vi "Generate Menu File.vi"(6 "Include Ancestor Palette ?":bool, 7 "Overwrite Always":bool, 8 "error in (no error)":errorcluster, 10 "Palette Fiole List":T7, 11 "Library as Project item":refnum<vi>) -> (0 "error out":errorcluster, 2 "palette data":T1={"display name"="", "view format"=0, "palette width"=4, "items"=[], "256 color icon"=bytes[0], "B&W color icon"=bytes[0], "help information"={"help tag"="", "help file path "=path ""}, "palette description"="", "synchronize information"={"synchronize with directory"=FALSE, "synchronize directory path"=path ""}} {"view format" items=["Icons", "Text", "Icons and Text"]}, 3 "Palette file path":path)   [LabVIEW 2012, in "Palette Generation.lvlib"]
doc: "This VI does most of the hard work, creating a palette file type def structure based on a list of project items that should belong in a virtual folder."
uses:
  Palette Generation.lvlib
  TypeDefs/Palette Fiole List.ctl
  <vilib>/Palette API/Palette Menu/Public Type Define/Palette Data.ctl
  <vilib>/Palette API/Palette Menu/Public Type Define/View Format.ctl
  <vilib>/Palette API/Palette Menu/Public Type Define/Items.ctl
  <vilib>/Palette API/Palette Menu/Public Type Define/Item.ctl
  <vilib>/Palette API/Palette Menu/Public Type Define/Help Info.ctl
  <vilib>/Palette API/Palette Menu/Public Type Define/Synchronize Info.ctl
  <vilib>/Palette API/Palette Menu/Public Type Define/Palette type.ctl
  <userlib>/_OpenG.lib/file/file.llb/File Exists - Scalar__ogtk.vi
  <userlib>/_OpenG.lib/file/file.llb/Strip Path Extension - String__ogtk.vi
  <userlib>/_OpenG.lib/file/file.llb/Convert File Extension (String)__ogtk.vi
  <userlib>/_OpenG.lib/file/file.llb/Strip Path Extension - Path__ogtk.vi
  <vilib>/regexp/Match Regular Expression.xnode
  <vilib>/Palette API/Palette Menu/Palette Menu.lvlib
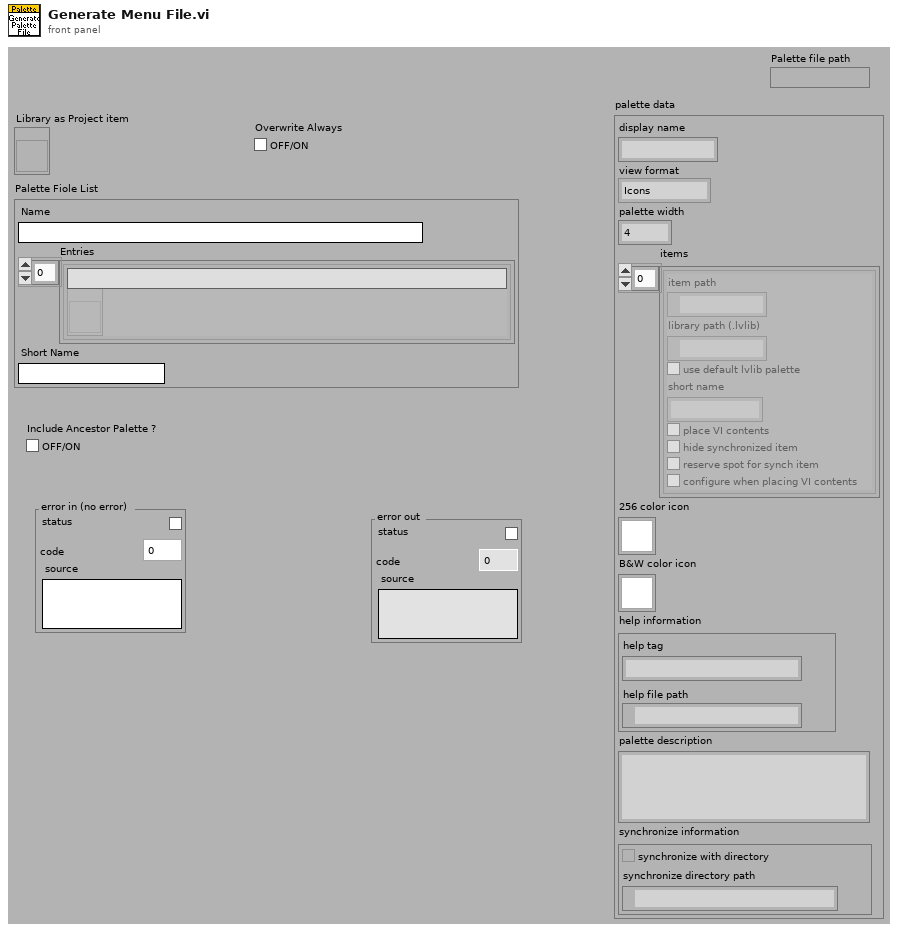
[diagram p1: front panel]
types:
  T1 = typedef "Palette Menu.lvlib/Palette Data.ctl" = cluster{"display name":string, "view format":T2, "palette width":i16, "items":T3, "256 color icon":picture, "B&W color icon":picture, "help information":T5, "palette description":string, "synchronize information":T6}
  T2 = typedef "Palette Menu.lvlib/View Format.ctl" = u16
  T3 = typedef "Palette Menu.lvlib/Items.ctl" = T4[]
  T4 = typedef "Palette Menu.lvlib/Item.ctl" = cluster{"item path":path, "library path (.lvlib)":path, "use default lvlib palette":bool, "short name":string, "place VI contents":bool, "hide synchronized item":bool, "reserve spot for synch item":bool, "configure when placing VI contents":bool}
  T5 = typedef "Palette Menu.lvlib/Help Info.ctl" = cluster{"help tag":string, "help file path ":path}
  T6 = typedef "Palette Menu.lvlib/Synchronize Info.ctl" = cluster{"synchronize with directory":bool, "synchronize directory path":path}
  T7 = typedef "Palette Generation.lvlib/Palette Fiole List.ctl" = cluster{"Name":string, "Entries":cluster{string, refnum<vi>}[], "Short Name":string}
  T8 = typedef "Palette Menu.lvlib/Palette type.ctl" = i32
  T9 = typedef "imagedata.ctl" = cluster{"image type":i32, "image depth":i32, "image":u8[], "mask":u8[], "colors":u32[], "Rectangle":cluster{"left":i16, "top":i16, "right":i16, "bottom":i16}}
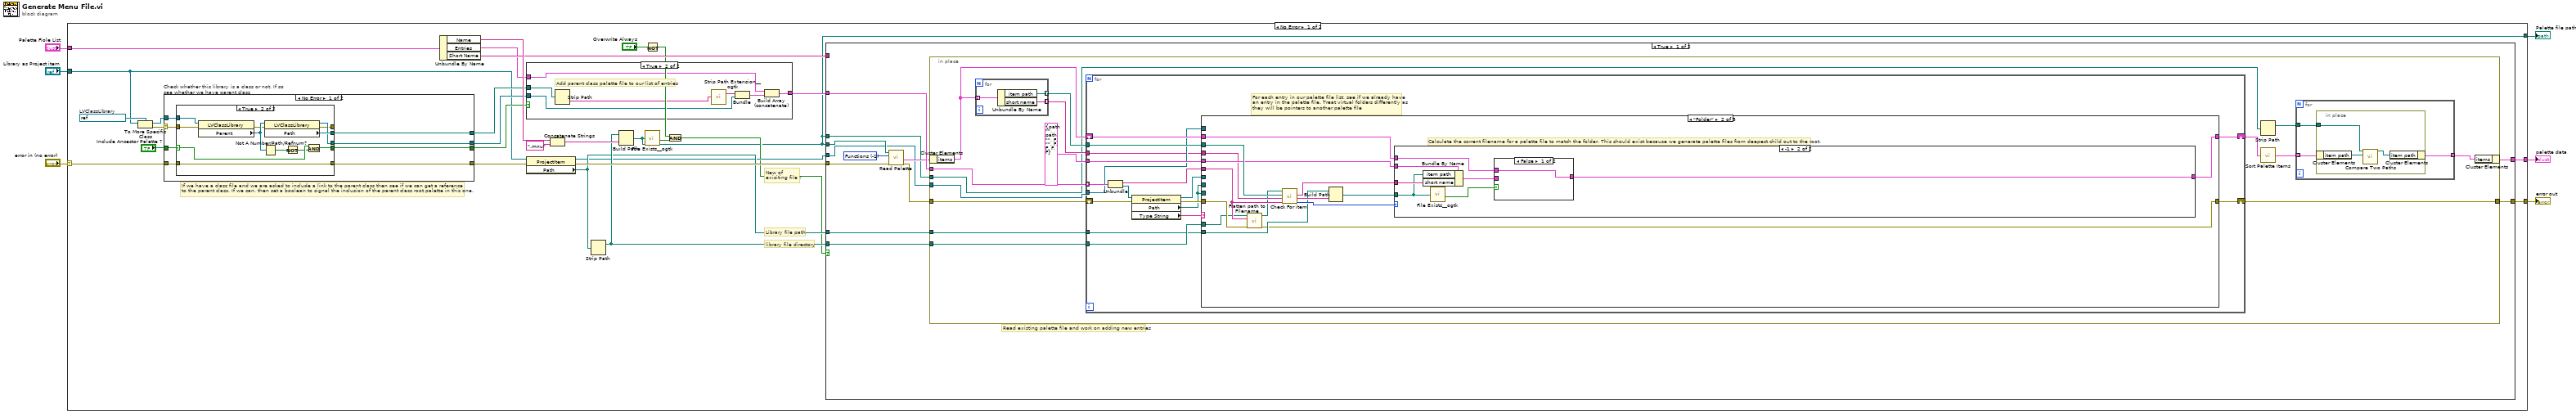
[diagram p0: block diagram]
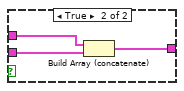
[diagram p7: hidden frame]
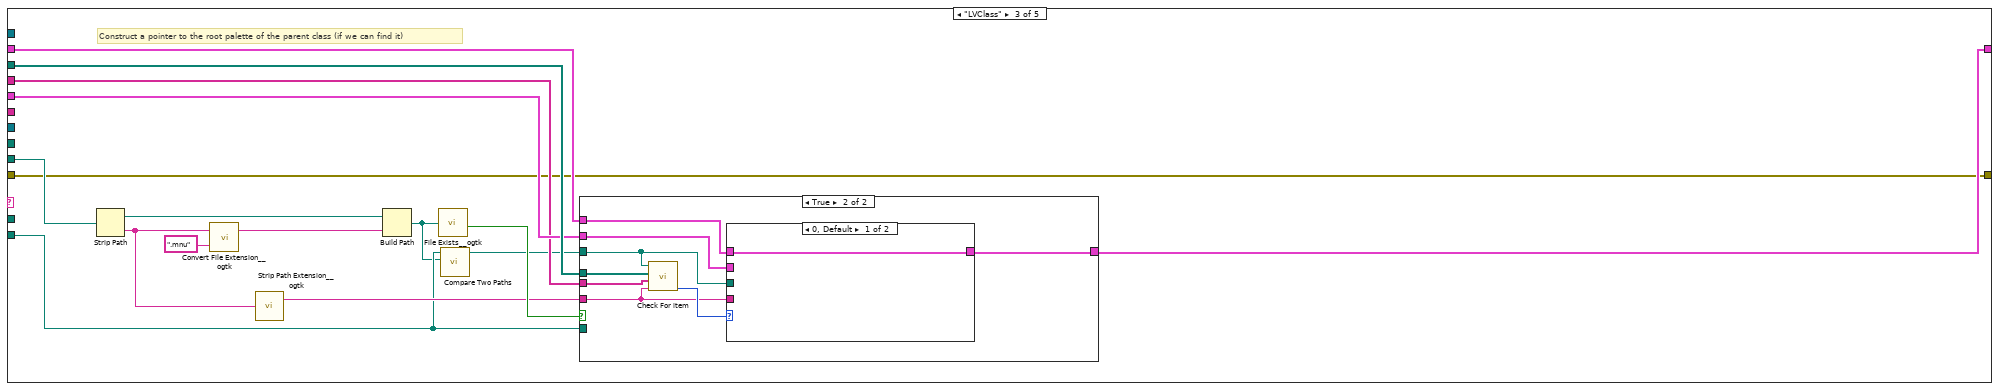
[diagram p8: hidden frame]
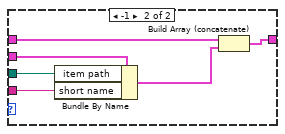
[diagram p10: hidden frame]
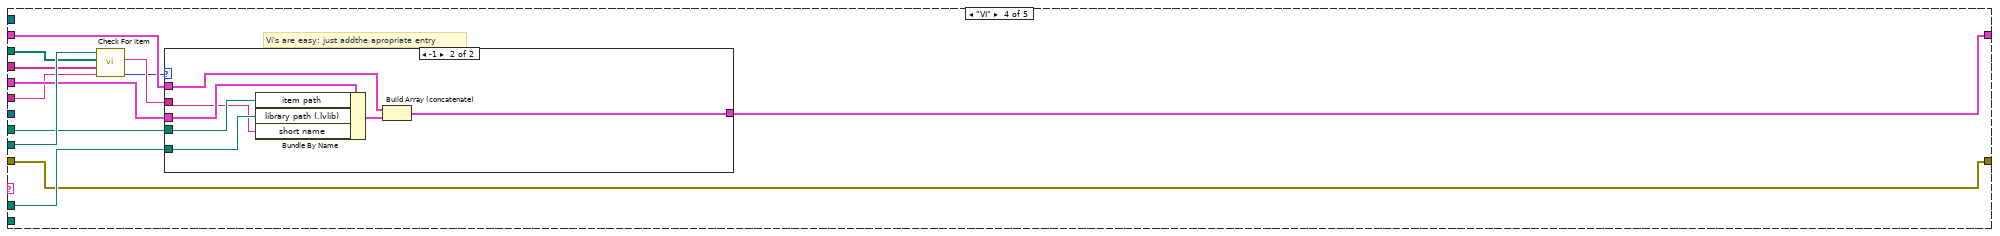
[diagram p11: hidden frame]
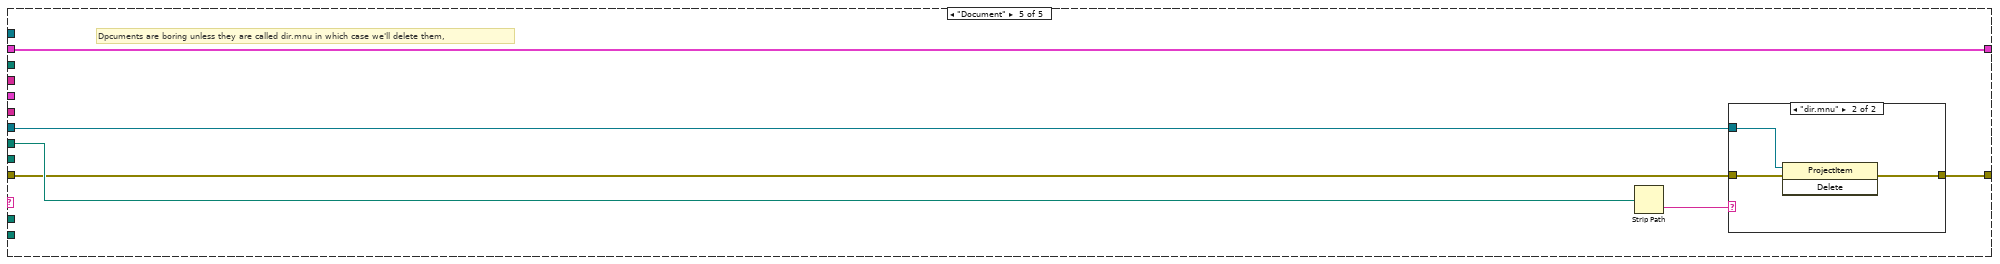
[diagram p13: hidden frame]
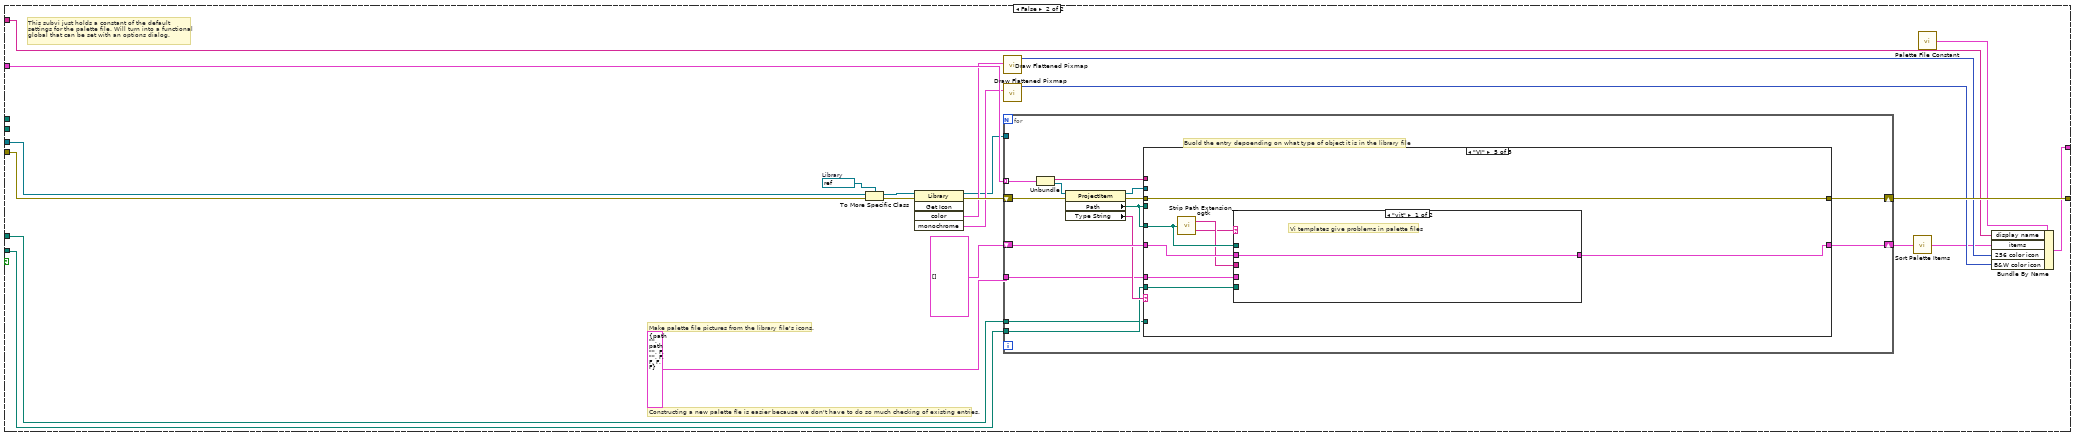
[diagram p15: hidden frame]
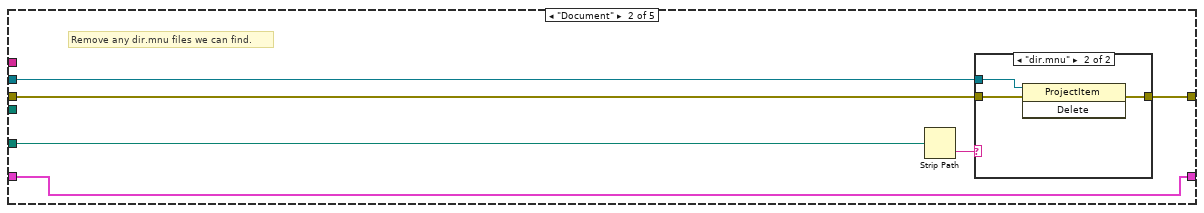
[diagram p17: hidden frame]
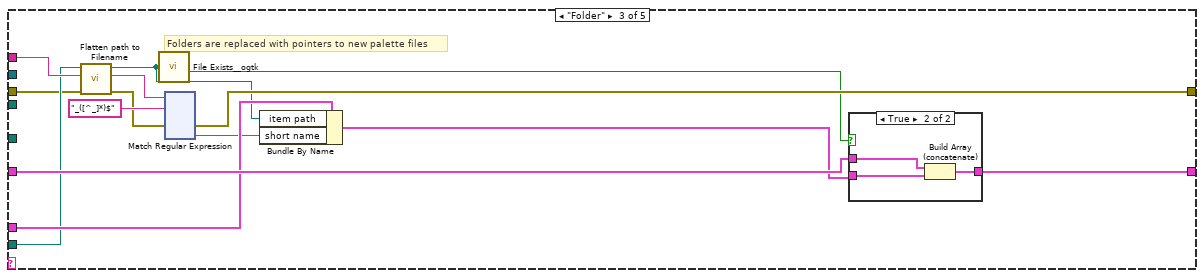
[diagram p19: hidden frame]
diagram:
  n1 = case shown="No Error" "error in (no error)" {
    selector: "error in (no error)" -> [w18 w425]
    tunnel: [w27 w425] -> w6
    tunnel: "Palette Fiole List" -> [w34 _]
    tunnel: "Library as Project item" -> [w9 _]
    tunnel: [w24 _] -> w2
    tunnel: [w7 _] -> w1
    frame No Error {
      w19 = refnum<vi> refnum  # LVClassLibrary
      # "New of\nexisiting file ?"
      # "library file directory"
      # "Library file path"
      # "If we have a class file and we are asked to include a link to the parent class then see if we can get a reference\nto the parent class. If we can, then set a boolean to signal the inclusion of the parent class root palette in this one."
      n2 = To More Specific Class(target class=w19, reference=w9) -> (specific class reference=w16:refnum<vi>, error out=w17:errorcluster)  [unwired: 1 in]
      n3 = case "Check whether this library is a class or not. If so see whether we have parent class" shown="No Error" w17 {
        selector: w17 -> [w49 _]
        tunnel: w18 -> [w43 w65]
        tunnel: w16 -> [w50 _]
        tunnel: [w47 _] -> w10
        tunnel: [w48 _] -> w11
        tunnel: [w46 w65] -> w15
        tunnel: [w44 _] -> w14
        tunnel: "Include Ancestor Palette ?" -> [w45 _]
        frame No Error {
          n4 = case shown="True" w45 {
            selector: w45 -> [w51 w60]
            tunnel: w50 -> [_ w64]
            tunnel: w49 -> [w52 w63]
            tunnel: [_ w62] -> w48
            tunnel: [_ w61] -> w47
            tunnel: [w52 w54] -> w46
            tunnel: [w51 w59] -> w44
            tunnel: w43 -> [_ w54]
            tunnel: [_ w53] -> _
            frame False {
            }
            frame True {
              n5 = property class="LVClassLibrary"(reference=w64, error in=w63) -> (error out=w55:errorcluster, "Parent"=w58:refnum<vi>)  [unwired: 1 out]
              n6 = Not A Number/Path/Refnum?(number/path/refnum=w58) -> (NaN/Path/Refnum?=w57:bool)
              n7 = property class="LVClassLibrary"(reference=w58, error in=w55) -> (reference out=w61:refnum<vi>, error out=w53:errorcluster, "Path"=w62:path)
              n8 = Not(x=w57) -> (.not. x?=w56:bool)
              n9 = And(x=w60, y=w56) -> (x .and. y?=w59:bool)
            }
          }
        }
        frame Error {
        }
      }
      n10 = Unbundle By Name(w34) -> ("Name"=w25:string, "Entries"=w12:cluster{string, refnum<vi>}[], "Short Name"=w23:string)
      n11 = case shown="True" w14 {
        tunnel: [w35 w41] -> w13
        tunnel: w12 -> [w35 w42]
        tunnel: w11 -> [_ w39]
        tunnel: w10 -> [_ w36]
        frame False {
        }
        frame True {
          # "Add parent class palette file to our list of entries"
          n12 = Strip Path(path=w39) -> (name=w40:string)  [unwired: 1 out]
          n13 = call-poly <userlib>:"Strip Path Extension__ogtk.vi"("path"=w40) -> ("root"=w37:string)  [unwired: 1 out]
          n14 = Bundle("root"=w37, "Parent"=w36) -> (w38:cluster{"root":string, "Parent":refnum<vi>})  [unwired: 1 out]
          n15 = Build Array (concatenate)(w42, w38) -> (w41:cluster{"root":string, "Parent":refnum<vi>}[])
        }
      }
      n16 = property class="ProjectItem"(reference=w9, error in=w15) -> (reference out=w26:refnum<vi>, error out=w30:errorcluster, "Path"=w28:path)
      n17 = Concatenate Strings(w25, ".mnu" ("string")) -> (w32:string)
      n18 = Strip Path(path=w28) -> (stripped path=w29:path)  [unwired: 1 out]
      n19 = Build Path(base path=w29, name or relative path=w32) -> (appended path=w7:path)
      n20 = call-poly <userlib>:"File Exists__ogtk.vi"("file path"=w7) -> ("exists"=w31:bool)  [unwired: 6 in, 1 out]
      n21 = Not(x="Overwrite Always") -> (.not. x?=w20:bool)
      n22 = And(x=w20, y=w31) -> (x .and. y?=w22:bool)
      n23 = case shown="True" w22 {
        tunnel: w7 -> [w77 _]
        tunnel: w30 -> [w75 w224]
        tunnel: w13 -> [w74 w233]
        tunnel: w29 -> [w72 w231]
        tunnel: w28 -> [w71 w230]
        tunnel: [w70 w229] -> w27
        tunnel: [w68 w226] -> w24
        tunnel: w26 -> [w67 w223]
        tunnel: w23 -> [_ w217]
        tunnel: w7 -> [w66 _]
        frame True {
          w76 = T8 -1 items=["Functions"=-1, "Controls"=-2] ("palette type")
          # "Read existing palette file and work on adding new entries"
          n24 = call <vilib>:"Read Palette.vi"("error in (no error)"=w75, "palette type"=w76, "palette path"=w77) -> ("error out"=w73:errorcluster, "palette data"=w69:T1)  [unwired: 1 in, 6 out]
          n25 = in-place {
            in-place-border: w74 -> [w92]
            in-place-border: w73 -> [w91]
            in-place-border: w72 -> [w89]
            in-place-border: w71 -> [w88]
            in-place-border: [w87] -> w70
            in-place-border: w67 -> [w86]
            in-place-border: w66 -> [w81]
            n26 = in-place-cluster #1(w69) -> ("items"=w85:T3)
            n27 = for {
              tunnel: w85 -> [w101] mode=indexing
              tunnel: [w100] -> w84 mode=indexing
              tunnel: [w99] -> w83 mode=indexing
              n28 = Unbundle By Name(w101) -> ("item path"=w100:path, "short name"=w99:string)
            }
            n29 = for {
              tunnel: w92 -> [w118] mode=indexing
              shift-right: [w107] -> w87
              shift-left: w91 -> [w116]
              tunnel: w84 -> [w115]
              shift-right: [w113] -> w82
              shift-left: w85 -> [w114]
              tunnel: T4 {"item path"=path "", "library path (.lvlib)"=path "", "use default lvlib palette"=FALSE, "short name"="", "place VI contents"=FALSE, "hide synchronized item"=FALSE, "reserve spot for synch item"=FALSE, "configure when placing VI contents"=FALSE} ("Items") -> [w110]
              tunnel: w89 -> [w109]
              tunnel: w88 -> [w108]
              tunnel: w86 -> [w104]
              tunnel: w83 -> [w102]
              # "For each entry in our palette file list, see if we already have\nan entry in the palette file. Treat virtual folders differently as\nthey will be pointers to another palette file"
              n30 = Unbundle(w118) -> ("root"=w111:string, "Parent"=w117:refnum<vi>)
              n31 = property class="ProjectItem"(reference=w117, error in=w116) -> (reference out=w103:refnum<vi>, error out=w106:errorcluster, "Path"=w105:path, "Type String"=w112:string)
              n32 = case shown="\"Folder\"" w112 {
                selector: w112 -> [w120 _ _ _ _]
                tunnel: w105 -> [w119 _ w160 w193 _]
                tunnel: w115 -> [_ w137 w165 w192 _]
                tunnel: w114 -> [w122 w134 w163 w191 w204]
                tunnel: [w122 w135 w164 w190 w204] -> w113
                tunnel: w111 -> [_ w127 _ w186 _]
                tunnel: w110 -> [_ w133 w162 w189 _]
                tunnel: w109 -> [_ w123 _ w187 _]
                tunnel: w108 -> [_ w128 w152 _ _]
                tunnel: [w121 w125 w154 w185 w203] -> w107
                tunnel: w106 -> [w121 w126 w154 w185 w205]
                tunnel: w105 -> [_ _ _ w188 w206]
                tunnel: w104 -> [_ _ _ _ _]
                tunnel: w103 -> [_ _ _ _ w202]
                tunnel: w102 -> [_ w131 w161 w184 _]
                frame "False", Default {
                  # "Ignore anything we don't recognise"
                  n33 = stacked-sequence {
                    tunnel: w120 -> [_]
                    tunnel: w119 -> [_]
                    frame #0 {
                    }
                  }
                }
                frame "Folder" {
                  # "Calculate the corrent filename for a palette file to match the folder. This should exist because we generate palette files from deepest child out to the root."
                  n34 = call "Flatten path to Filename.vi"("error in (no error)"=w126, "Virtual Folder's Virtual Path"=w127, "Library Base Path"=w123) -> ("error out"=w125:errorcluster, "Palette Path"=w124:path)  [unwired: 6 out]
                  n35 = call "Check For item.vi"("This Name"=w127, "short names"=w131, "item paths"=w137, "This Path"=w124) -> ("index of element"=w136:i32, "Flattened Name"=w129:string, "Short Name"=w132:string)  [unwired: 5 out]
                  n36 = Build Path(base path=w128, name or relative path=w129) -> (appended path=w130:path)
                  n37 = case shown="-1" w136 {
                    tunnel: [w138 w144] -> w135
                    tunnel: w134 -> [w138 w145]
                    tunnel: w133 -> [_ w143]
                    tunnel: w130 -> [_ w140]
                    tunnel: w132 -> [_ w142]
                    frame 0, Default {
                    }
                    frame -1 {
                      n38 = Bundle By Name(cluster=w143, "item path"=w140, "short name"=w142) -> (w141:T4)
                      n39 = call-poly <userlib>:"File Exists__ogtk.vi"("file path"=w140) -> ("exists"=w139:bool)  [unwired: 6 in, 1 out]
                      n40 = case shown="False" w139 {
                        tunnel: w145 -> [w146 w149]
                        tunnel: [w146 w148] -> w144
                        tunnel: w141 -> [_ w147]
                        frame False {
                        }
                        frame True {
                          n41 = Build Array (concatenate)(w149, w147) -> (w148:T3)
                        }
                      }
                    }
                  }
                }
                frame "LVClass" {
                  # "Construct a pointer to the root palette of the parent class (if we can find it)"
                  n42 = Strip Path(path=w160) -> (stripped path=w157:path, name=w156:string)
                  n43 = call-poly <userlib>:"Convert File Extension__ogtk.vi"("new ending (none)"=".mnu", "file name"=w156) -> ("new filename"=w158:string)  [unwired: 1 out]
                  n44 = call-poly <userlib>:"Strip Path Extension__ogtk.vi"("path"=w156) -> ("root"=w153:string)  [unwired: 1 out]
                  n45 = Build Path(base path=w157, name or relative path=w158) -> (appended path=w151:path)
                  n46 = call-poly <userlib>:"File Exists__ogtk.vi"("file path"=w151) -> ("exists"=w155:bool)  [unwired: 6 in, 1 out]
                  n47 = call <vilib>:"Compare Two Paths.vi"("Path 2"=w151, "Path 1"=w152) -> ("Relative Path from 1 to 2"=w150:path)  [unwired: 1 in, 8 out]
                  n48 = case shown="True" w155 {
                    tunnel: w165 -> [_ w174]
                    tunnel: [w166 w172] -> w164
                    tunnel: w163 -> [w166 w171]
                    tunnel: w162 -> [_ w170]
                    tunnel: w161 -> [_ w169]
                    tunnel: w152 -> [_ _]
                    tunnel: w153 -> [_ w167]
                    tunnel: w150 -> [_ w168]
                    frame False {
                    }
                    frame True {
                      n49 = call "Check For item.vi"("This Name"=w167, "short names"=w169, "item paths"=w174, "This Path"=w168) -> ("index of element"=w173:i32)  [unwired: 7 out]
                      n50 = case shown="0, Default" w173 {
                        tunnel: [w175 w180] -> w172
                        tunnel: w171 -> [w175 w181]
                        tunnel: w170 -> [_ w179]
                        tunnel: w168 -> [_ w178]
                        tunnel: w167 -> [_ w177]
                        frame 0, Default {
                        }
                        frame -1 {
                          n51 = Bundle By Name(cluster=w179, "item path"=w178, "short name"=w177) -> (w176:T4)
                          n52 = Build Array (concatenate)(w181, w176) -> (w180:T3)
                        }
                      }
                    }
                  }
                }
                frame "VI" {
                  # "Vi's are easy: just addthe apropriate entry"
                  n53 = call "Check For item.vi"("This Name"=w186, "short names"=w184, "item paths"=w192, "This Path"=w193) -> ("index of element"=w182:i32, "Short Name"=w183:string)  [unwired: 6 out]
                  n54 = case shown="-1" w182 {
                    tunnel: w191 -> [w194 w201]
                    tunnel: [w194 w200] -> w190
                    tunnel: w189 -> [_ w199]
                    tunnel: w188 -> [_ w197]
                    tunnel: w187 -> [_ w196]
                    tunnel: w183 -> [_ w195]
                    frame 0, Default {
                    }
                    frame -1 {
                      n55 = Bundle By Name(cluster=w199, "item path"=w197, "library path (.lvlib)"=w196, "short name"=w195) -> (w198:T4)
                      n56 = Build Array (concatenate)(w201, w198) -> (w200:T3)
                    }
                  }
                }
                frame "Document" {
                  # "Dpcuments are boring unless they are called dir.mnu in which case we'll delete them,"
                  n57 = Strip Path(path=w206) -> (name=w207:string)  [unwired: 1 out]
                  n58 = case shown="\"dir.mnu\"" w207 {
                    tunnel: w205 -> [w208 w211]
                    tunnel: w202 -> [_ w210]
                    tunnel: [w208 w209] -> w203
                    frame "False", Default {
                    }
                    frame "dir.mnu" {
                      n59 = invoke class="ProjectItem" method="Delete"(reference=w210, error in=w211) -> (error out=w209:errorcluster)  [unwired: 1 in, 2 out]
                    }
                  }
                }
              }
            }
            n60 = Strip Path(path=w81) -> (stripped path=w80:path)  [unwired: 1 out]
            n61 = call "Sort Palette Items.vi"("Array 2"=w82) -> ("Array"=w79:T4[])
            n62 = for {
              tunnel: w79 -> [w95] mode=indexing
              tunnel: w80 -> [w94]
              tunnel: [w93] -> w78 mode=indexing
              n63 = in-place {
                in-place-border: w94 -> [w97]
                n64 = in-place-cluster #2(w95) -> ("item path"=w98:path)
                n65 = call <vilib>:"Compare Two Paths.vi"("Path 2"=w98, "Path 1"=w97) -> ("Relative Path from 1 to 2"=w96:path)  [unwired: 1 in, 8 out]
                n66 = in-place-cluster #2("item path"=w96) -> (w93:T4)
              }
            }
            n67 = in-place-cluster #1("items"=w78) -> (w68:T1)
          }
        }
        frame False {
          w222 = refnum<vi> refnum  # Library
          # "This subvi just holds a constant of the default\nsettings for the palette file. Will turn into a functional\nglobal that can be set with an options dialog."
          # "Make palette file pictures from the library file's icons."
          # "Constructing a new palette fle is easier because we don't have to do so much checking of existing entries."
          n68 = To More Specific Class(target class=w222, reference=w223, error in=w224) -> (specific class reference=w221:refnum<vi>, error out=w220:errorcluster)
          n69 = invoke class="Library" method="Get Icon"(reference=w221, error in=w220) -> (reference out=w214:refnum<vi>, error out=w225:errorcluster, "color"=w219:T9, "monochrome"=w216:T9)  [unwired: 3 in, 1 out]
          n70 = call <vilib>:"Draw Flattened Pixmap.vi"("image data"=w219) -> ("new picture"=w218:picture)  [unwired: 1 in, 7 out]
          n71 = call <vilib>:"Draw Flattened Pixmap.vi"("image data"=w216) -> ("new picture"=w215:picture)  [unwired: 1 in, 7 out]
          n72 = for {
            tunnel: w233 -> [w247] mode=indexing
            shift-right: [w238] -> w229
            shift-left: w225 -> [w245]
            shift-right: [w243] -> w213
            shift-left: T4[] [] -> [w244]
            tunnel: T4 {"item path"=path "", "library path (.lvlib)"=path "", "use default lvlib palette"=FALSE, "short name"="", "place VI contents"=FALSE, "hide synchronized item"=FALSE, "reserve spot for synch item"=FALSE, "configure when placing VI contents"=FALSE} ("Items") -> [w241]
            tunnel: w231 -> [w240]
            tunnel: w230 -> [w239]
            tunnel: w214 -> [_]
            # "Buold the entry depoending on what type of object it is in the library file"
            n73 = Unbundle(w247) -> ("root"=w235:string, "Parent"=w246:refnum<vi>)
            n74 = property class="ProjectItem"(reference=w246, error in=w245) -> (reference out=w234:refnum<vi>, error out=w237:errorcluster, "Path"=w236:path, "Type String"=w242:string)
            n75 = case shown="\"VI\"" w242 {
              selector: w242 -> [w249 _ _ _ _]
              tunnel: w236 -> [_ _ _ w396 _]
              tunnel: w244 -> [w251 w253 w274 w405 w414]
              tunnel: [w251 w253 w275 w406 w413] -> w243
              tunnel: w241 -> [_ _ w273 w404 w412]
              tunnel: w240 -> [_ _ w266 _ w411]
              tunnel: w239 -> [_ _ _ w395 _]
              tunnel: [w250 w254 w270 w402 w408] -> w238
              tunnel: w237 -> [w250 w255 w265 w402 w408]
              tunnel: w236 -> [w248 w257 _ _ w410]
              tunnel: w235 -> [_ _ w268 _ _]
              tunnel: w234 -> [_ w252 _ _ _]
              frame "False", Default {
                # "An unknown type"
                n76 = stacked-sequence {
                  tunnel: w249 -> [_]
                  tunnel: w248 -> [_]
                  frame #0 {
                  }
                }
              }
              frame "Document" {
                # "Remove any dir.mnu files we can find."
                n77 = Strip Path(path=w257) -> (name=w256:string)  [unwired: 1 out]
                n78 = case shown="\"dir.mnu\"" w256 {
                  tunnel: w255 -> [w258 w261]
                  tunnel: w252 -> [_ w260]
                  tunnel: [w258 w259] -> w254
                  frame "False", Default {
                  }
                  frame "dir.mnu" {
                    n79 = invoke class="ProjectItem" method="Delete"(reference=w260, error in=w261) -> (error out=w259:errorcluster)  [unwired: 1 in, 2 out]
                  }
                }
              }
              frame "Folder" {
                # "Folders are replaced with pointers to new palette files"
                n80 = call "Flatten path to Filename.vi"("error in (no error)"=w265, "Virtual Folder's Virtual Path"=w268, "Library Base Path"=w266) -> ("error out"=w264:errorcluster, "result string"=w267:string, "Palette Path"=w263:path)  [unwired: 5 out]
                n81 = call-poly <userlib>:"File Exists__ogtk.vi"("file path"=w263) -> ("exists"=w262:bool)  [unwired: 6 in, 1 out]
                n82 = xnode "Match Regular Expression"("input string"=w267, "regular expression"="_([^_]*)$", "error in"=w264) -> ("error out"=w270:errorcluster, "submatch 1"=w269:string)  [unwired: 1 in, 6 out]
                n83 = Bundle By Name(cluster=w273, "item path"=w263, "short name"=w269) -> (w272:T4)
                n84 = case shown="True" w262 {
                  tunnel: [w276 w279] -> w275
                  tunnel: w274 -> [w276 w278]
                  tunnel: w272 -> [_ w277]
                  frame False {
                  }
                  frame True {
                    n85 = Build Array (concatenate)(w278, w277) -> (w279:T4[])
                  }
                }
              }
              frame "LVClass" {
                # "Classes are replaced with pointers to the root palette file if it exists. This is called when the parent class link is required."
                n86 = Strip Path(path=w396) -> (stripped path=w399:path, name=w400:string)
                n87 = call-poly <userlib>:"Strip Path Extension__ogtk.vi"("path"=w400) -> ("root"=w393:string)  [unwired: 1 out]
                n88 = call-poly <userlib>:"Convert File Extension__ogtk.vi"("new ending (none)"=".mnu", "file name"=w400) -> ("new filename"=w398:string)  [unwired: 1 out]
                n89 = Build Path(base path=w399, name or relative path=w398) -> (appended path=w401:path)
                n90 = call-poly <userlib>:"File Exists__ogtk.vi"("file path"=w401) -> ()  [unwired: 6 in, 2 out]
                n91 = call <vilib>:"Compare Two Paths.vi"("Path 2"=w401, "Path 1"=w395) -> ("Relative Path from 1 to 2"=w394:path)  [unwired: 1 in, 8 out]
                n92 = Bundle By Name(cluster=w404, "item path"=w394, "short name"=w393) -> (w403:T4)
                n93 = Build Array (concatenate)(w405, w403) -> (w406:T4[])
              }
              frame "VI" {
                n94 = call-poly <userlib>:"Strip Path Extension__ogtk.vi"("path"=w410) -> ("root"=w409:string, "extension"=w407:string)
                n95 = case shown="\"vit\"" w407 {
                  tunnel: w414 -> [w415 w424]
                  tunnel: [w415 w423] -> w413
                  tunnel: w412 -> [_ w422]
                  tunnel: w411 -> [_ w421]
                  tunnel: w410 -> [_ w418]
                  tunnel: w409 -> [_ w417]
                  frame "vit" {
                    # "Vi templates give problems in palette files"
                  }
                  frame "True", Default {
                    # "A VI is stragihtforward"
                    n96 = String To Path(string=w417) -> (path=w416:path)
                    n97 = Strip Path(path=w416) -> (name=w419:string)  [unwired: 1 out]
                    n98 = Bundle By Name(cluster=w422, "item path"=w418, "library path (.lvlib)"=w421, "short name"=w419) -> (w420:T4)
                    n99 = Build Array (concatenate)(w424, w420) -> (w423:T4[])
                  }
                }
              }
            }
          }
          n100 = call "Sort Palette Items.vi"("Array 2"=w213) -> ("Array"=w212:T4[])
          n101 = call "Palette File Constant.vi"() -> ("palette data"=w227:T1)
          n102 = Bundle By Name(cluster=w227, "display name"=w217, "items"=w212, "256 color icon"=w218, "B&W color icon"=w215) -> (w226:T1)
        }
      }
    }
    frame Error {
    }
  }
  "error out" <- w6
  "palette data" <- w2
  "Palette file path" <- w1
